vi "MQTT Property (Developer Helper).vi"() -> ()   [LabVIEW 2019, in "KoRE-MQTT.lvlib"]
doc: "Copyright (c) 2025 KoRElibs.com\nSPDX-License-Identifier: EUPL-1.2\n\nThis VI is licensed under the European Union Public License (EUPL) Version 1.2. You may use this VI unmodified in proprietary works. If you distribute a modified version of this file, the modified file must be released under the EUPL-1.2. Full license: https://joinup.ec.europa.eu/asset/eupl/eupl/1.2/"
uses:
  KoRE-MQTT.lvlib
  MQTT Property - AUTH.ctl
  MQTT Property - CONNECT.ctl
  MQTT Property - DISCONNECT.ctl
  MQTT Property - PUBCOMP.ctl
  MQTT Property - Will.ctl
  MQTT Property - CONNACK.ctl
  MQTT Property - PUBACK.ctl
  MQTT Property - PUBREC.ctl
  MQTT Property - PUBLISH.ctl
  MQTT Property - UNSUBACK.ctl
  MQTT Property - PUBREL.ctl
  MQTT Property - SUBACK.ctl
  MQTT Property - SUBSCRIBE.ctl
  MQTT Property - UNSUBSCRIBE.ctl
  MQTT Property - GENERIC.ctl
  MQTT Property Type.ctl
panel:
  in  "General MQTT Property":T1 {"Property" items=[" Name                              "=0, " Payload Format Indicator          "=1, " Message Expiry Interval           "=2, " Content Type                      "=3, " Response Topic                    "=8, " Correlation Data                  "=9, " Subscription Identifier           "=11, " Session Expiry Interval           "=17, " Assigned Client Identifier        "=18, " Server Keep Alive                 "=19, " Authentication Method             "=21, " Authentication Data               "=22, " Request Problem Information       "=23, " Will Delay Interval               "=24, " Request Response Information      "=25, " Response Information              "=26, " Server Reference                  "=28, " Reason String                     "=31, " Receive Maximum                   "=33, " Topic Alias Maximum               "=34, " Topic Alias                       "=35, " Maximum QoS                       "=36, " Retain Available                  "=37, " User Property (\"key:value\")       "=38, " Maximum Packet Size               "=39, " Wildcard Subscription Available   "=40, " Subscription Identifier Available "=41, " Shared Subscription Available     "=42]}
  in  "UNSUBSCRIBE Property":T3 {"Property" items=[" User Property (\"key:value\")       "=38]}
  in  "SUBSCRIBE Property":T4 {"Property" items=[" Subscription Identifier           "=11, " User Property (\"key:value\")       "=38]}
  in  "SUBACK Property":T5 {"Property" items=[" Reason String                     "=31, " User Property (\"key:value\")       "=38]}
  in  "PUBREL Property":T6 {"Property" items=[" Reason String                     "=31, " User Property (\"key:value\")       "=38]}
  in  "UNSUBACK Property":T7 {"Property" items=[" Reason String                     "=31, " User Property (\"key:value\")       "=38]}
  in  "PUBLISH Property":T8 {"Property" items=[" Payload Format Indicator          "=1, " Message Expiry Interval           "=2, " Content Type                      "=3, " Response Topic                    "=8, " Correlation Data                  "=9, " Subscription Identifier           "=11, " Topic Alias                       "=35, " User Property (\"key:value\")       "=38]}
  in  "PUBREC Property":T9 {"Property" items=[" Reason String                     "=31, " User Property (\"key:value\")       "=38]}
  in  "PUBACK Property":T10 {"Property" items=[" Reason String                     "=31, " User Property (\"key:value\")       "=38]}
  in  "CONNACK Property":T11 {"Property" items=[" Session Expiry Interval           "=17, " Assigned Client Identifier        "=18, " Server Keep Alive                 "=19, " Authentication Method             "=21, " Authentication Data               "=22, " Response Information              "=26, " Server Reference                  "=28, " Reason String                     "=31, " Receive Maximum                   "=33, " Topic Alias Maximum               "=34, " Maximum QoS                       "=36, " Retain Available                  "=37, " User Property (\"key:value\")       "=38, " Maximum Packet Size               "=39, " Wildcard Subscription Available   "=40, " Subscription Identifier Available "=41, " Shared Subscription Available     "=42]}
  in  "Will Property":T12 {"Property" items=[" Payload Format Indicator          "=1, " Message Expiry Interval           "=2, " Content Type                      "=3, " Response Topic                    "=8, " Correlation Data                  "=9, " Will Delay Interval               "=24, " User Property (\"key:value\")       "=38]}
  in  "PUBCOMP Property":T13 {"Property" items=[" Reason String                     "=31, " User Property (\"key:value\")       "=38]}
  in  "DISCONNECT Property":T14 {"Property" items=[" Session Expiry Interval           "=17, " Server Reference                  "=28, " Reason String                     "=31, " User Property (\"key:value\")       "=38]}
  in  "CONNECT Property":T15 {"Property" items=[" Session Expiry Interval           "=17, " Authentication Method             "=21, " Authentication Data               "=22, " Request Problem Information       "=23, " Request Response Information      "=25, " Receive Maximum                   "=33, " Topic Alias Maximum               "=34, " User Property (\"key:value\")       "=38, " Maximum Packet Size               "=39]}
  in  "AUTH Property":T16 {"Property" items=[" Authentication Method             "=21, " Authentication Data               "=22, " Reason String                     "=31, " User Property (\"key:value\")       "=38]}
  # "All Properties"
  # "Client Properties"
  # "Server Properties"
  # "Client/Server Properties"
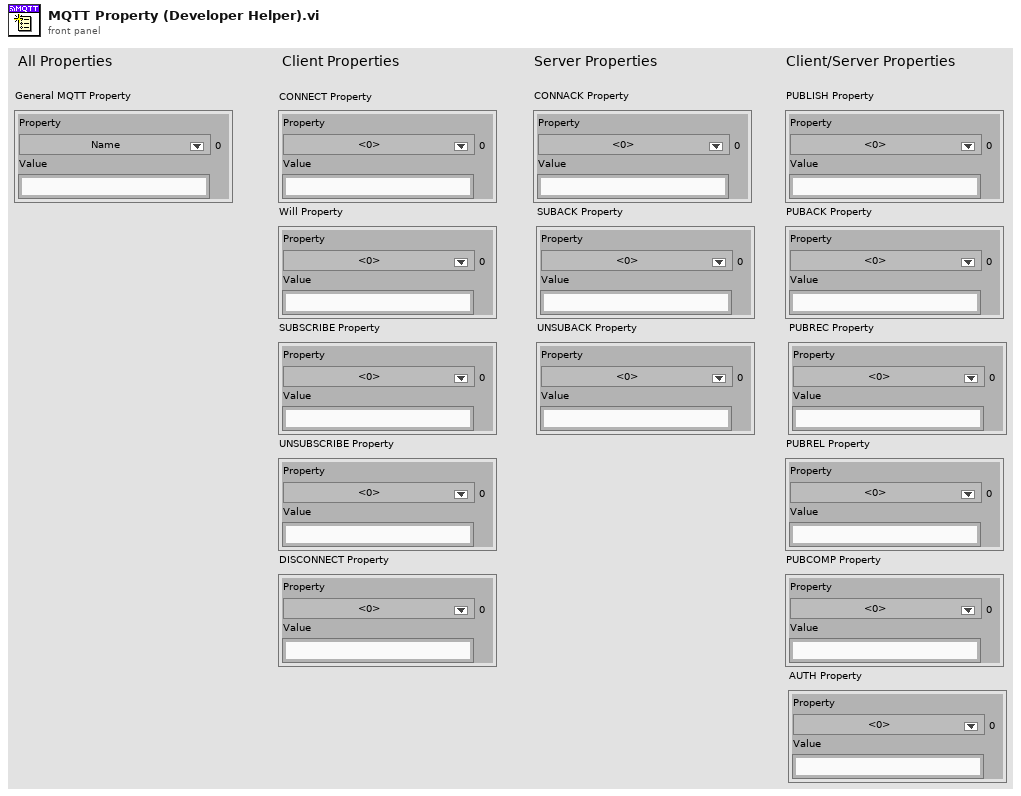
[diagram p1: front panel]
types:
  T1 = typedef "KoRE-MQTT.lvlib/MQTT Property - GENERIC.ctl" = cluster{"Property":T2, "Value":string}
  T2 = typedef "KoRE-MQTT.lvlib/MQTT Property Type.ctl" = u8
  T3 = typedef "KoRE-MQTT.lvlib/MQTT Property - UNSUBSCRIBE.ctl" = cluster{"Property":u8, "Value":string}
  T4 = typedef "KoRE-MQTT.lvlib/MQTT Property - SUBSCRIBE.ctl" = cluster{"Property":u8, "Value":string}
  T5 = typedef "KoRE-MQTT.lvlib/MQTT Property - SUBACK.ctl" = cluster{"Property":u8, "Value":string}
  T6 = typedef "KoRE-MQTT.lvlib/MQTT Property - PUBREL.ctl" = cluster{"Property":u8, "Value":string}
  T7 = typedef "KoRE-MQTT.lvlib/MQTT Property - UNSUBACK.ctl" = cluster{"Property":u8, "Value":string}
  T8 = typedef "KoRE-MQTT.lvlib/MQTT Property - PUBLISH.ctl" = cluster{"Property":u8, "Value":string}
  T9 = typedef "KoRE-MQTT.lvlib/MQTT Property - PUBREC.ctl" = cluster{"Property":u8, "Value":string}
  T10 = typedef "KoRE-MQTT.lvlib/MQTT Property - PUBACK.ctl" = cluster{"Property":u8, "Value":string}
  T11 = typedef "KoRE-MQTT.lvlib/MQTT Property - CONNACK.ctl" = cluster{"Property":u8, "Value":string}
  T12 = typedef "KoRE-MQTT.lvlib/MQTT Property - Will.ctl" = cluster{"Property":u8, "Value":string}
  T13 = typedef "KoRE-MQTT.lvlib/MQTT Property - PUBCOMP.ctl" = cluster{"Property":u8, "Value":string}
  T14 = typedef "KoRE-MQTT.lvlib/MQTT Property - DISCONNECT.ctl" = cluster{"Property":u8, "Value":string}
  T15 = typedef "KoRE-MQTT.lvlib/MQTT Property - CONNECT.ctl" = cluster{"Property":u8, "Value":string}
  T16 = typedef "KoRE-MQTT.lvlib/MQTT Property - AUTH.ctl" = cluster{"Property":u8, "Value":string}
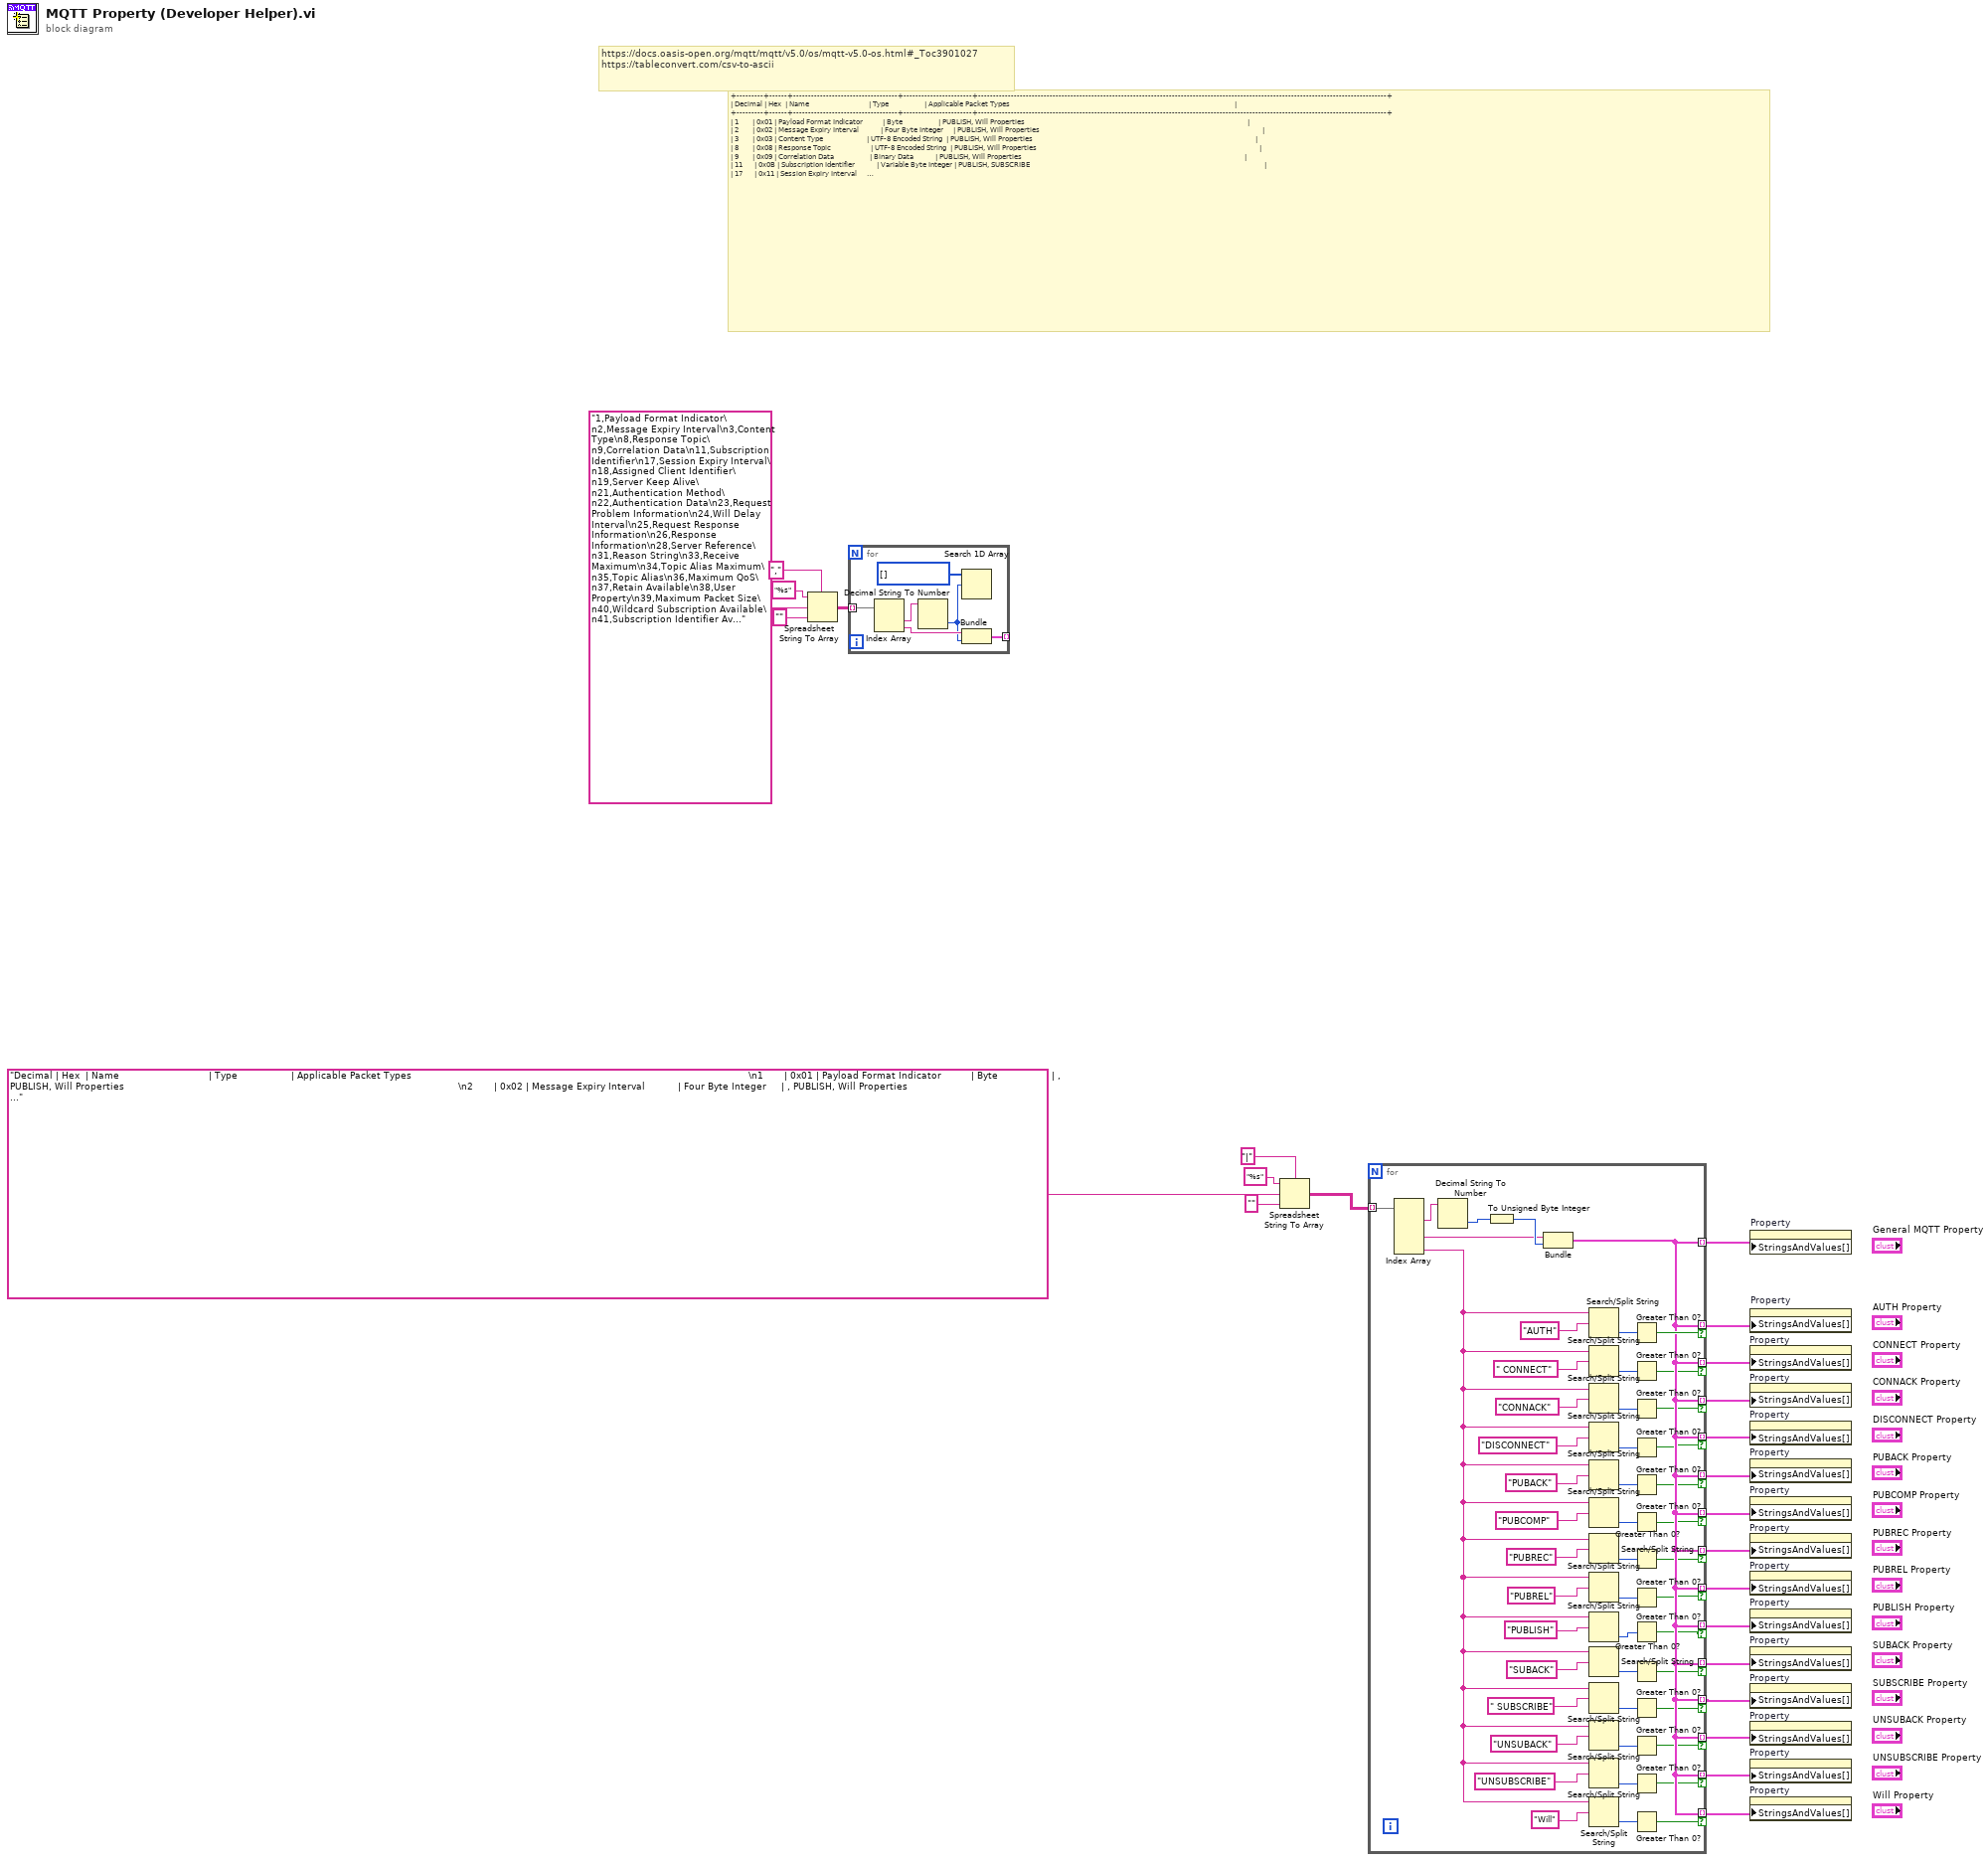
[diagram p0: block diagram]
diagram:
  # "https://docs.oasis-open.org/mqtt/mqtt/v5.0/os/mqtt-v5.0-os.html#_Toc3901027\nhttps://tableconvert.com/csv-to-ascii"
  # "+---------+------+-----------------------------------+-----------------------+-----------------------------------------------------------------------------------------------------------------------------------------+\n| Decimal | Hex  | Name                              | Type                  | Applicable Packet Types                                                                                                                 |\n+---------+------+-----------------------------------+-----------------------+-----------------------------------------------------------------------------------------------------------------------------------------+\n| 1       | 0x01 | Payload Format Indicator          | Byte                  | PUBLISH, Will Properties                                                                                                                |\n| 2       | 0x02 | Message Expiry Interval           | Four Byte Integer     | PUBLISH, Will Properties                                                                                                                |\n| 3       | 0x03 | Content Type                      | UTF-8 Encoded String  | PUBLISH, Will Properties                                                                                                                |\n| 8       | 0x08 | Response Topic                    | UTF-8 Encoded String  | PUBLISH, Will Properties                                                                                                                |\n| 9       | 0x09 | Correlation Data                  | Binary Data           | PUBLISH, Will Properties                                                                                                                |\n| 11      | 0x0B | Subscription Identifier           | Variable Byte Integer | PUBLISH, SUBSCRIBE                                                                                                                      |\n| 17      | 0x11 | Session Expiry Interval           | Four Byte Integer     | CONNECT, CONNACK, DISCONNECT                                                                                                            |\n| 18      | 0x12 | Assigned Client Identifier        | UTF-8 Encoded String  | CONNACK                                                                                                                                 |\n| 19      | 0x13 | Server Keep Alive                 | Two Byte Integer      | CONNACK                                                                                                                                 |\n| 21      | 0x15 | Authentication Method             | UTF-8 Encoded String  | CONNECT, CONNACK, AUTH                                                                                                                  |\n| 22      | 0x16 | Authentication Data               | Binary Data           | CONNECT, CONNACK, AUTH                                                                                                                  |\n| 23      | 0x17 | Request Problem Information       | Byte                  | CONNECT                                                                                                                                 |\n| 24      | 0x18 | Will Delay Interval               | Four Byte Integer     | Will Properties                                                                                                                         |\n| 25      | 0x19 | Request Response Information      | Byte                  | CONNECT                                                                                                                                 |\n| 26      | 0x1A | Response Information              | UTF-8 Encoded String  | CONNACK                                                                                                                                 |\n| 28      | 0x1C | Server Reference                  | UTF-8 Encoded String  | CONNACK, DISCONNECT                                                                                                                     |\n| 31      | 0x1F | Reason String                     | UTF-8 Encoded String  | CONNACK, PUBACK, PUBREC, PUBREL, PUBCOMP, SUBACK, UNSUBACK, DISCONNECT, AUTH                                                            |\n| 33      | 0x21 | Receive Maximum                   | Two Byte Integer      | CONNECT, CONNACK                                                                                                                        |\n| 34      | 0x22 | Topic Alias Maximum               | Two Byte Integer      | CONNECT, CONNACK                                                                                                                        |\n| 35      | 0x23 | Topic Alias                       | Two Byte Integer      | PUBLISH                                                                                                                                 |\n| 36      | 0x24 | Maximum QoS                       | Byte                  | CONNACK                                                                                                                                 |\n| 37      | 0x25 | Retain Available                  | Byte                  | CONNACK                                                                                                                                 |\n| 38      | 0x26 | User Property                     | UTF-8 String Pair     | CONNECT, CONNACK, PUBLISH, Will Properties, PUBACK, PUBREC, PUBREL, PUBCOMP, SUBSCRIBE, SUBACK, UNSUBSCRIBE, UNSUBACK, DISCONNECT, AUTH |\n| 39      | 0x27 | Maximum Packet Size               | Four Byte Integer     | CONNECT, CONNACK                                                                                                                        |\n| 40      | 0x28 | Wildcard Subscription Available   | Byte                  | CONNACK                                                                                                                                 |\n| 41      | 0x29 | Subscription Identifier Available | Byte                  | CONNACK                                                                                                                                 |\n| 42      | 0x2A | Shared Subscription Available     | Byte                  | CONNACK                                                                                                                                 |\n+---------+------+-----------------------------------+-----------------------+-----------------------------------------------------------------------------------------------------------------------------------------+"
  n1 = Spreadsheet String To Array(delimiter (Tab)=",", format string="%s", spreadsheet string="1,Payload Format Indicator\n2,Message Expiry Interval\n3,Content Type\n8,Response Topic\n9,Correlation Data\n11,Subscription Identifier\n17,Session Expiry Interval\n18,Assigned Client Identifier\n19,Server Keep Alive\n21,Authentication Method\n22,Authentication Data\n23,Request Problem Information\n24,Will Delay Interval\n25,Request Response Information\n26,Response Information\n28,Server Reference\n31,Reason String\n33,Receive Maximum\n34,Topic Alias Maximum\n35,Topic Alias\n36,Maximum QoS\n37,Retain Available\n38,User Property\n39,Maximum Packet Size\n40,Wildcard Subscription Available\n41,Subscription Identifier Available\n42,Shared Subscription Available", array type (2D Dbl)="") -> (array=w21:string[][])
  n2 = for {
    tunnel: w21 -> [w31] mode=indexing
    tunnel: [w28] -> _ mode=indexing
    n3 = Index Array(array=w31) -> (element #1=w30:string, element #2=w29:string)  [unwired: 2 in]
    n4 = Decimal String To Number(string=w30) -> (number=w27:i32)  [unwired: 2 in, 1 out]
    n5 = Search 1D Array(1D array=i32[] [], element=w27) -> ()  [unwired: 1 in, 1 out]
    n6 = Bundle(w29, w27) -> (w28:cluster{string, i32})  [unwired: 1 in]
  }
  n7 = Spreadsheet String To Array(delimiter (Tab)="|", format string="%s", spreadsheet string="Decimal | Hex  | Name                              | Type                  | Applicable Packet Types                                                                                                                 \n1       | 0x01 | Payload Format Indicator          | Byte                  | , PUBLISH, Will Properties                                                                                                                \n2       | 0x02 | Message Expiry Interval           | Four Byte Integer     | , PUBLISH, Will Properties                                                                                                                \n3       | 0x03 | Content Type                      | UTF-8 Encoded String  | , PUBLISH, Will Properties                                                                                                                \n8       | 0x08 | Response Topic                    | UTF-8 Encoded String  | , PUBLISH, Will Properties                                                                                                                \n9       | 0x09 | Correlation Data                  | Binary Data           | , PUBLISH, Will Properties                                                                                                                \n11      | 0x0B | Subscription Identifier           | Variable Byte Integer | , PUBLISH, SUBSCRIBE                                                                                                                      \n17      | 0x11 | Session Expiry Interval           | Four Byte Integer     | , CONNECT, CONNACK, DISCONNECT                                                                                                            \n18      | 0x12 | Assigned Client Identifier        | UTF-8 Encoded String  | , CONNACK                                                                                                                                 \n19      | 0x13 | Server Keep Alive                 | Two Byte Integer      | , CONNACK                                                                                                                                 \n21      | 0x15 | Authentication Method             | UTF-8 Encoded String  | , CONNECT, CONNACK, AUTH                                                                                                                  \n22      | 0x16 | Authentication Data               | Binary Data           | , CONNECT, CONNACK, AUTH                                                                                                                  \n23      | 0x17 | Request Problem Information       | Byte                  | , CONNECT                                                                                                                                 \n24      | 0x18 | Will Delay Interval               | Four Byte Integer     | , Will Properties                                                                                                                         \n25      | 0x19 | Request Response Information      | Byte                  | , CONNECT                                                                                                                                 \n26      | 0x1A | Response Information              | UTF-8 Encoded String  | , CONNACK                                                                                                                                 \n28      | 0x1C | Server Reference                  | UTF-8 Encoded String  | , CONNACK, DISCONNECT                                                                                                                     \n31      | 0x1F | Reason String                     | UTF-8 Encoded String  | , CONNACK, PUBACK, PUBREC, PUBREL, PUBCOMP, SUBACK, UNSUBACK, DISCONNECT, AUTH                                                            \n33      | 0x21 | Receive Maximum                   | Two Byte Integer      | , CONNECT, CONNACK                                                                                                                        \n34      | 0x22 | Topic Alias Maximum               | Two Byte Integer      | , CONNECT, CONNACK                                                                                                                        \n35      | 0x23 | Topic Alias                       | Two Byte Integer      | , PUBLISH                                                                                                                                 \n36      | 0x24 | Maximum QoS                       | Byte                  | , CONNACK                                                                                                                                 \n37      | 0x25 | Retain Available                  | Byte                  | , CONNACK                                                                                                                                 \n38      | 0x26 | User Property (\"key:value\")       | UTF-8 String Pair     | , CONNECT, CONNACK, PUBLISH, Will Properties, PUBACK, PUBREC, PUBREL, PUBCOMP, SUBSCRIBE, SUBACK, UNSUBSCRIBE, UNSUBACK, DISCONNECT, AUTH \n39      | 0x27 | Maximum Packet Size               | Four Byte Integer     | , CONNECT, CONNACK                                                                                                                        \n40      | 0x28 | Wildcard Subscription Available   | Byte                  | , CONNACK                                                                                                                                 \n41      | 0x29 | Subscription Identifier Available | Byte                  | , CONNACK                                                                                                                                 \n42      | 0x2A | Shared Subscription Available     | Byte                  | , CONNACK                                                                                                                                 \n", array type (2D Dbl)="") -> (array=w16:string[][])
  n8 = for {
    tunnel: w16 -> [w80] mode=indexing
    tunnel: [w47] -> w1 mode=indexing
    tunnel: [w47] -> w15 mode=indexing if=w76
    tunnel: [w47] -> w2 mode=indexing if=w45
    tunnel: [w47] -> w3 mode=indexing if=w44
    tunnel: [w47] -> w4 mode=indexing if=w43
    tunnel: [w47] -> w5 mode=indexing if=w42
    tunnel: [w47] -> w6 mode=indexing if=w41
    tunnel: [w47] -> w7 mode=indexing if=w40
    tunnel: [w47] -> w8 mode=indexing if=w39
    tunnel: [w47] -> w9 mode=indexing if=w38
    tunnel: [w47] -> w10 mode=indexing if=w37
    tunnel: [w47] -> w11 mode=indexing if=w36
    tunnel: [w47] -> w12 mode=indexing if=w35
    tunnel: [w47] -> w13 mode=indexing if=w34
    tunnel: [w47] -> w14 mode=indexing if=w46
    n9 = Index Array(array=w80) -> (element #1=w79:string, element #3=w32:string, element #5=w48:string)  [unwired: 5 in, 2 out]
    n10 = Decimal String To Number(string=w79) -> (number=w78:i32)  [unwired: 2 in, 1 out]
    n11 = To Unsigned Byte Integer(number=w78) -> (unsigned 8bit integer=w33:u8)
    n12 = Bundle(w32, w33) -> (w47:cluster{string, u8})  [unwired: 1 in]
    n13 = Search/Split String(string=w48, search string/char (-)="AUTH") -> (offset of match=w77:i32)  [unwired: 1 in, 2 out]
    n14 = Search/Split String(string=w48, search string/char (-)=" CONNECT") -> (offset of match=w74:i32)  [unwired: 1 in, 2 out]
    n15 = Search/Split String(string=w48, search string/char (-)="CONNACK") -> (offset of match=w72:i32)  [unwired: 1 in, 2 out]
    n16 = Search/Split String(string=w48, search string/char (-)="DISCONNECT") -> (offset of match=w70:i32)  [unwired: 1 in, 2 out]
    n17 = Search/Split String(string=w48, search string/char (-)="PUBACK") -> (offset of match=w68:i32)  [unwired: 1 in, 2 out]
    n18 = Search/Split String(string=w48, search string/char (-)="PUBCOMP") -> (offset of match=w66:i32)  [unwired: 1 in, 2 out]
    n19 = Search/Split String(string=w48, search string/char (-)="PUBREC") -> (offset of match=w64:i32)  [unwired: 1 in, 2 out]
    n20 = Search/Split String(string=w48, search string/char (-)="PUBREL") -> (offset of match=w62:i32)  [unwired: 1 in, 2 out]
    n21 = Search/Split String(string=w48, search string/char (-)="PUBLISH") -> (offset of match=w60:i32)  [unwired: 1 in, 2 out]
    n22 = Search/Split String(string=w48, search string/char (-)="SUBACK") -> (offset of match=w58:i32)  [unwired: 1 in, 2 out]
    n23 = Search/Split String(string=w48, search string/char (-)=" SUBSCRIBE") -> (offset of match=w56:i32)  [unwired: 1 in, 2 out]
    n24 = Search/Split String(string=w48, search string/char (-)="UNSUBACK") -> (offset of match=w55:i32)  [unwired: 1 in, 2 out]
    n25 = Search/Split String(string=w48, search string/char (-)="UNSUBSCRIBE") -> (offset of match=w53:i32)  [unwired: 1 in, 2 out]
    n26 = Search/Split String(string=w48, search string/char (-)="Will") -> (offset of match=w51:i32)  [unwired: 1 in, 2 out]
    n27 = Greater Than 0?(x=w77) -> (x > 0?=w76:bool)
    n28 = Greater Than 0?(x=w74) -> (x > 0?=w45:bool)
    n29 = Greater Than 0?(x=w72) -> (x > 0?=w44:bool)
    n30 = Greater Than 0?(x=w70) -> (x > 0?=w43:bool)
    n31 = Greater Than 0?(x=w68) -> (x > 0?=w42:bool)
    n32 = Greater Than 0?(x=w66) -> (x > 0?=w41:bool)
    n33 = Greater Than 0?(x=w64) -> (x > 0?=w40:bool)
    n34 = Greater Than 0?(x=w62) -> (x > 0?=w39:bool)
    n35 = Greater Than 0?(x=w60) -> (x > 0?=w38:bool)
    n36 = Greater Than 0?(x=w58) -> (x > 0?=w37:bool)
    n37 = Greater Than 0?(x=w56) -> (x > 0?=w36:bool)
    n38 = Greater Than 0?(x=w55) -> (x > 0?=w35:bool)
    n39 = Greater Than 0?(x=w53) -> (x > 0?=w34:bool)
    n40 = Greater Than 0?(x=w51) -> (x > 0?=w46:bool)
  }
  n41 = property on="Property" class="Ring (strict)"("StringsAndValues[]"=w1) -> ()  [unwired: 2 in, 2 out]
  n42 = property on="Property" class="Ring (strict)"("StringsAndValues[]"=w15) -> ()  [unwired: 2 in, 2 out]
  n43 = property on="Property" class="Ring (strict)"("StringsAndValues[]"=w2) -> ()  [unwired: 2 in, 2 out]
  n44 = property on="Property" class="Ring (strict)"("StringsAndValues[]"=w3) -> ()  [unwired: 2 in, 2 out]
  n45 = property on="Property" class="Ring (strict)"("StringsAndValues[]"=w4) -> ()  [unwired: 2 in, 2 out]
  n46 = property on="Property" class="Ring (strict)"("StringsAndValues[]"=w5) -> ()  [unwired: 2 in, 2 out]
  n47 = property on="Property" class="Ring (strict)"("StringsAndValues[]"=w6) -> ()  [unwired: 2 in, 2 out]
  n48 = property on="Property" class="Ring (strict)"("StringsAndValues[]"=w7) -> ()  [unwired: 2 in, 2 out]
  n49 = property on="Property" class="Ring (strict)"("StringsAndValues[]"=w8) -> ()  [unwired: 2 in, 2 out]
  n50 = property on="Property" class="Ring (strict)"("StringsAndValues[]"=w9) -> ()  [unwired: 2 in, 2 out]
  n51 = property on="Property" class="Ring (strict)"("StringsAndValues[]"=w10) -> ()  [unwired: 2 in, 2 out]
  n52 = property on="Property" class="Ring (strict)"("StringsAndValues[]"=w11) -> ()  [unwired: 2 in, 2 out]
  n53 = property on="Property" class="Ring (strict)"("StringsAndValues[]"=w12) -> ()  [unwired: 2 in, 2 out]
  n54 = property on="Property" class="Ring (strict)"("StringsAndValues[]"=w13) -> ()  [unwired: 2 in, 2 out]
  n55 = property on="Property" class="Ring (strict)"("StringsAndValues[]"=w14) -> ()  [unwired: 2 in, 2 out]
